vi "Open.vi"(8 "error in":errorcluster, 9 "parameters":variant, 10 "file path":path, 11 "repository in":refnum<class "SystemConfigRepo.lvclass">) -> (0 "error out":errorcluster, 2 "invalid?":bool, 3 "repository out":refnum<class "SystemConfigRepo.lvclass">)   [LabVIEW 2014, in "PL Framework Configuration Tool.lvlib" / "SystemConfigRepo.lvclass"]
doc: "Loads the saved information of the repo. If a module in the configuration cannot be found it is replaced by the Missing Plugin module in Configuration Editor\\Classes\\Missing Plugin.\n\nLicensed under the Apache License, Version 2.0 (the \"License\"); you may not use this file except in compliance with the License. You may obtain a copy of the License at http://www.apache.org/licenses/LICENSE-2.0\nUnless required by applicable law or agreed to in writing, software distributed under the License is distributed on an \"AS IS\" BASIS, WITHOUT WARRANTIES OR CONDITIONS OF ANY KIND, either express or implied. See the License for the specific language governing permissions and limitations under the License."
uses:
  SystemConfigRepo.lvclass
  <vilib>/NI/Configuration Framework/tree serializer/NISE_CEF_TreeSerializer.lvlib
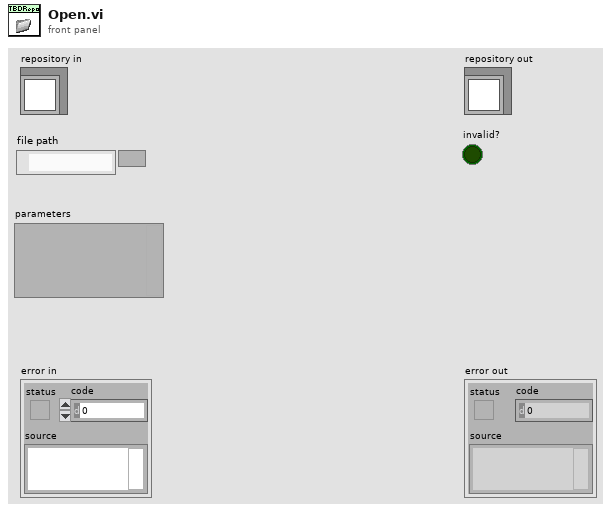
[diagram p1: front panel]
types:
  T1 = typedef "NISE_CEF_TreeSerializer.lvlib/base file format.ctl" = cluster{"version":string, "data":string}
  T2 = typedef "NISE_CEF_TreeSerializer.lvlib/flat hierarchy.ctl" = cluster{"hierarchy structure":T3, "instance data":T5[]}
  T3 = typedef "NISE_CEF_TreeSerializer.lvlib/full hierarchy.ctl" = cluster{"root":string, "hierarchy":T4[]}
  T4 = typedef "NISE_CEF_TreeSerializer.lvlib/hierarchy element.ctl" = cluster{"current node":string, "children":string[]}
  T5 = typedef "NISE_CEF_TreeSerializer.lvlib/instance data.ctl" = cluster{"ID":string, "Alias":string, "class":string, "version":string, "data":string}
  T6 = typedef "NISE_CEF_TreeSerializer.lvlib/memory hierarchy.ctl" = cluster{"hierarchy structure":T3, "instance data":refnum<class "NISE_CEF_serializable configuration.lvclass">[]}
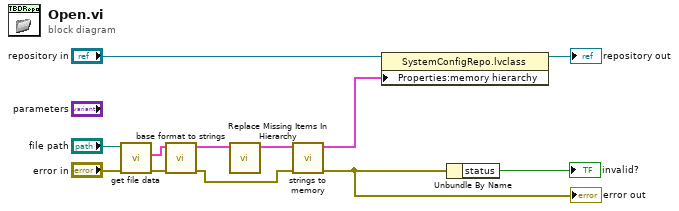
[diagram p0: block diagram]
diagram:
  n1 = call <vilib>:"get file data.vi"("error in"="error in", "Path"="file path") -> ("error out"=w11:errorcluster, "format"=w12:T1)  [unwired: 8 in]
  n2 = call <vilib>:"base format to strings.vi"("error in"=w11, "format"=w12) -> ("error out"=w1:errorcluster, "data"=w3:T2)  [unwired: 8 in]
  n3 = call "Replace Missing Items In Hierarchy.vi"("Flat Hierarchy"=w3) -> ("Flat Hierarchy"=w2:T2)  [unwired: 10 in]
  n4 = call <vilib>:"strings to memory.vi"("error in"=w1, "1.0.0"=w2) -> ("error out"=w5:errorcluster, "memory hierarchy"=w4:T6)  [unwired: 8 in]
  "error out" <- w5
  n5 = property class="SystemConfigRepo.lvclass"(reference="repository in", "Properties:memory hierarchy"=w4) -> (reference out=→"repository out":refnum<class "SystemConfigRepo.lvclass">)  [unwired: 1 in, 1 out]
  n6 = Unbundle By Name(w5) -> ("status"=→"invalid?":bool)
